vi "Timestamp to ISO 8601 UTC.vi"(8 "error in (no error)":errorcluster, 11 "Timestamp":timestamp) -> (0 "error out":errorcluster, 3 "ISO 8601 UTC":string)   [LabVIEW 2020, in "Time Management.lvlib"]
doc: "Formats a timestamp as an ISO 8601 string in UTC with milliseconds, for example 2025-10-06T13:02:11.250Z. The result does not depend on the Windows decimal-separator setting: the milliseconds are computed as an integer and formatted separately. A timestamp of 0 (the LabVIEW epoch) returns an empty string, which the storage layer uses for a running entry's End Time.\nA\nAGenerated by: Claude"
uses:
  Time Management.lvlib
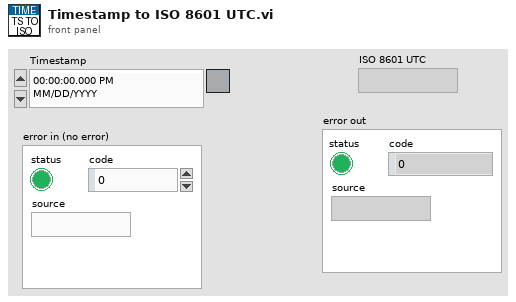
[diagram p1: front panel]
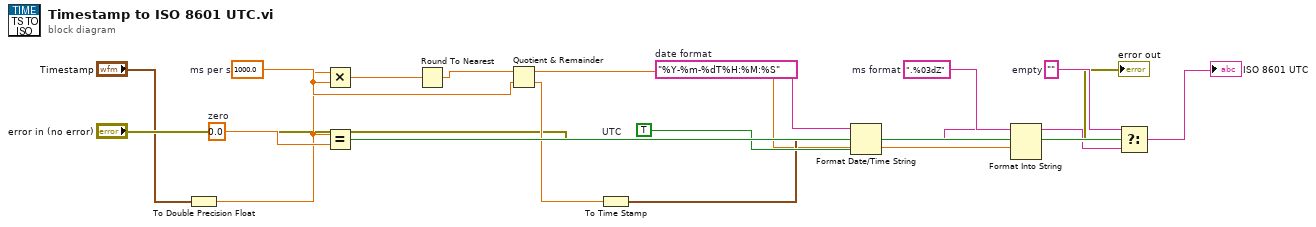
[diagram p0: block diagram]
diagram:
  w18 = ""  # empty
  w16 = 0.0  # zero
  w13 = ".%03dZ"  # ms format
  w11 = TRUE  # UTC
  w10 = "%Y-%m-%dT%H:%M:%S"  # date format
  w4 = 1000.0  # ms per s
  n1 = To Double Precision Float(number="Timestamp") -> (double precision float=w3:dbl)
  n2 = Multiply(x=w3, y=w4) -> (x*y=w5:dbl)
  n3 = Equal?(x=w3, y=w16) -> (x = y?=w17:bool)
  n4 = Round To Nearest(number=w5) -> (nearest integer value=w6:dbl)
  n5 = Quotient & Remainder(x=w6, y=w4) -> (x-y*floor(x/y)=w7:dbl, floor(x/y)=w8:dbl)
  n6 = To Time Stamp(1:w8) -> (0:w9:timestamp)
  n7 = Format Date/Time String(time format string (%c)=w10, seconds (now)=w9, UTC format=w11) -> (date/time string=w12:string)
  n8 = Format Into String(format string=w13, initial string=w12, error in="error in (no error)", w7) -> (resulting string=w14:string, error out=→"error out":errorcluster)
  n9 = Select(t=w18, s=w17, f=w14) -> (s? t:f=→"ISO 8601 UTC":string)
